vi "Proto Parser.vi"(8 "error in (no error)":errorcluster, 10 "Import Paths":path[](array[path]), 11 ".proto file path":path) -> (0 "error out":errorcluster, 1 "gRPC Method Parameters":T5[](array[typedef]), 2 "gRPC Enum Parameters":T1[](array[typedef]), 3 "gRPC Message Parameters":T2[](array[typedef]), 4 "Serialized Proto":string)   [LabVIEW 2019, in "gRPC Template Creation Utility.lvlib"]
uses:
  gRPC Template Creation Utility.lvlib
  TypeDefs/RPC Method Parameters.ctl
  TypeDefs/Message Metadata (Scripting).ctl
  TypeDefs/Message Element Metadata (Scripting).ctl
  TypeDefs/Message Element Type.ctl
  TypeDefs/Enum Metadata (Scripting).ctl
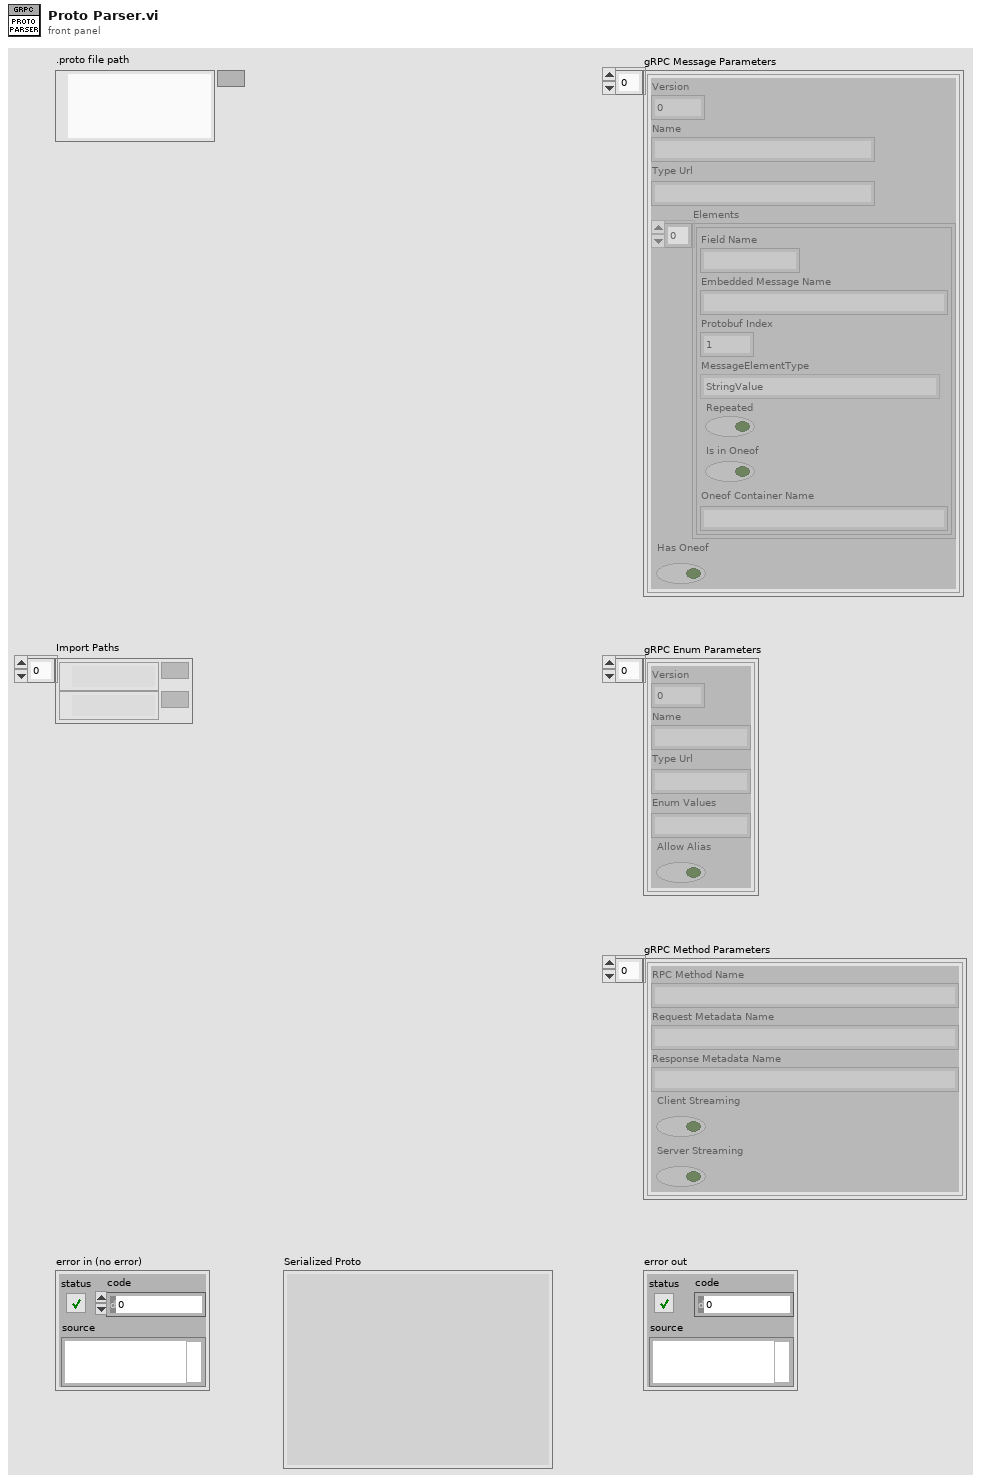
[diagram p1: front panel]
types:
  T1 = typedef "gRPC Template Creation Utility.lvlib/Enum Metadata (Scripting).ctl" = cluster{"Version":i32, "Name":string, "Type Url":string, "Enum Values":string, "Allow Alias":bool}
  T2 = typedef "gRPC Template Creation Utility.lvlib/Message Metadata (Scripting).ctl" = cluster{"Version":i32, "Name":string, "Type Url":string, "Elements":T3[], "Has Oneof":bool}
  T3 = typedef "gRPC Template Creation Utility.lvlib/Message Element Metadata (Scripting).ctl" = cluster{"Field Name":string, "Embedded Message Name":string, "Protobuf Index":i32, "MessageElementType":T4, "Repeated":bool, "Is in Oneof":bool, "Oneof Container Name":string}
  T4 = typedef "gRPC Template Creation Utility.lvlib/Message Element Type.ctl" = enum32{"Int32Value", "FloatValue", "DoubleValue", "BoolValue", "StringValue", "MessageValue", "Int64Value", "UInt32Value", "UInt64Value", "EnumValue", "Bytes", "Fixed64", "Fixed32", "SFixed64", "SFixed32", "SInt64", "SInt32"}
  T5 = typedef "gRPC Template Creation Utility.lvlib/RPC Method Parameters.ctl" = cluster{"RPC Method Name":string, "Request Metadata Name":string, "Response Metadata Name":string, "Client Streaming":bool, "Server Streaming":bool}
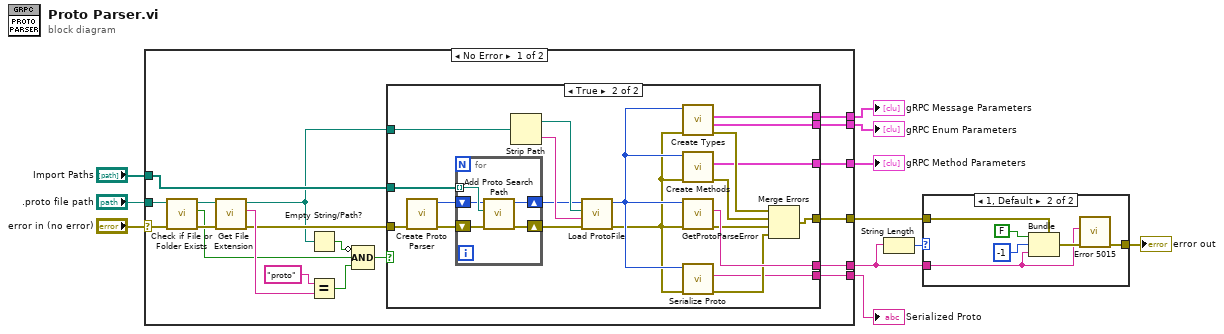
[diagram p0: block diagram]
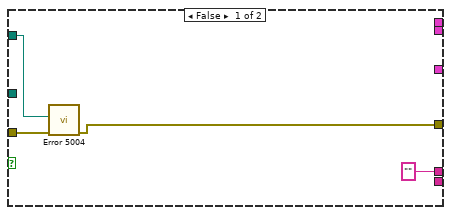
[diagram p3: hidden frame]
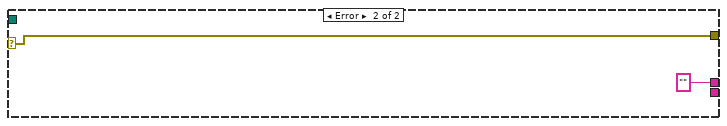
[diagram p4: hidden frame]
diagram:
  n1 = case shown="No Error" "error in (no error)" {
    selector: "error in (no error)" -> [w27 w62]
    tunnel: ".proto file path" -> [w28 _]
    tunnel: [w30 _] -> w11
    tunnel: [w29 w62] -> w5
    tunnel: [w19 _] -> w8
    tunnel: "Import Paths" -> [w18 _]
    tunnel: [w17 "" ("Error Message")] -> w3
    tunnel: [w16 _] -> w2
    tunnel: [w15 _] -> w1
    frame No Error {
      n2 = call <vilib>:"Check if File or Folder Exists.vi"("error in (no error)"=w27, "path"=w28) -> ("error out"=w26:errorcluster, "file or folder exists?"=w14:bool, "dup path"=w25:path)  [unwired: 7 in]
      n3 = call <vilib>:"Get File Extension.vi"("error in (no error)"=w26, "file"=w25) -> ("error out"=w20:errorcluster, "lowercase file extension"=w24:string, "dup file"=w12:path)  [unwired: 5 in, 2 out]
      n4 = Empty String/Path?(string/path=w12) -> (empty?=w13:bool)
      n5 = Equal?(x="proto", y=w24) -> (x = y?=w22:bool)
      n6 = Compound Arithmetic op=AND(invert w13, w14, w22) -> (w21:bool)
      n7 = case shown="True" w21 {
        tunnel: [_ w35] -> w30
        tunnel: [w33 w53] -> w29
        tunnel: w12 -> [w32 w55]
        tunnel: w20 -> [w34 w51]
        tunnel: [_ w36] -> w19
        tunnel: w18 -> [_ w50]
        tunnel: ["" ("Error Message") w46] -> w17
        tunnel: [_ w37] -> w16
        tunnel: [_ w39] -> w15
        frame False {
          n8 = call "Error 5004.vi"("error in (no error)"=w34, "Proto file path"=w32) -> ("error out"=w33:errorcluster)  [unwired: 9 in]
        }
        frame True {
          n9 = call "Create Proto Parser.vi"("error in (no error)"=w51) -> ("error out"=w49:errorcluster, "protoFile ref out"=w45:u64)  [unwired: 9 in]
          n10 = for {
            tunnel: w50 -> [w60] mode=indexing
            shift-right: [w56] -> w38
            shift-left: w45 -> [w57]
            shift-right: [w58] -> w48
            shift-left: w49 -> [w59]
            n11 = call "Add Proto Search Path.vi"("error in (no error)"=w59, "Search Path"=w60, "protoFile ref in"=w57) -> ("error out"=w58:errorcluster, "protoFile ref out"=w56:u64)  [unwired: 7 in]
          }
          n12 = Strip Path(path=w55) -> (stripped path=w47:path, name=w52:string)
          n13 = call "Load ProtoFile.vi"("protoFile ref in"=w38, "File Base path"=w47, "File Name"=w52, "error in (no error)"=w48) -> ("protoFile ref out"=w42:u64, "error out"=w41:errorcluster)  [unwired: 5 in]
          n14 = call "Create Types.vi"("error in (no error)"=w41, "protoFile ref in"=w42) -> ("error out"=w44:errorcluster, "Enum Parameters"=w37:T1[], "Message Parameters"=w36:T2[])  [unwired: 6 in, 1 out]
          n15 = call "Create Methods.vi"("error in (no error)"=w41, "protoFile ref in"=w42) -> ("error out"=w54:errorcluster, "Method Parameters"=w35:T5[])  [unwired: 7 in, 1 out]
          n16 = call "GetProtoParseError.vi"("error in (no error)"=w41, "Protofile ref in"=w42) -> ("error out"=w43:errorcluster, "Error Message"=w46:string)  [unwired: 7 in, 1 out]
          n17 = call "Serialize Proto.vi"("protoFile ref in"=w42, "error in (no error)"=w41) -> ("outBuffer"=w39:string, "error out"=w40:errorcluster)  [unwired: 6 in, 1 out]
          n18 = Merge Errors(w44, w54, w43, w40) -> (w53:errorcluster)
        }
      }
    }
    frame Error {
    }
  }
  "gRPC Method Parameters" <- w11
  "gRPC Message Parameters" <- w8
  "gRPC Enum Parameters" <- w2
  "Serialized Proto" <- w1
  n19 = String Length(string=w3) -> (length=w6:i32)
  n20 = case shown="1, Default" w6 {
    tunnel: w5 -> [w63 w69]
    tunnel: [w63 w64] -> w4
    tunnel: w3 -> [_ w65]
    frame 0 {
    }
    frame 1, Default {
      n21 = Bundle(cluster=w69, "status"=FALSE, "code"=-1, "source"=w65) -> (w66:errorcluster)
      n22 = call "Error 5015.vi"("error in (no error)"=w66, "Additional Error text"=w65) -> ("error out"=w64:errorcluster)  [unwired: 9 in]
    }
  }
  "error out" <- w4
